vi "Create.vi"   [LabVIEW 2018, in "Toolkit.lvlib" / "Agent.lvclass"]
doc: "Creates a new Agent object that represents a libssh2lv shared library Agent struct. This VI must be called, or executed, before using any other Agent-related VIs. This VI allocates memory within the libssh2lv shared library that must be explicitly deallocated, or freed, at the end of the application using the <B>Destroy</B> VI to avoid memory leaks or running Out-of-Memory (OOM) on a resource contrained system.\n\nAn Agent object represents a connection to a SSH-agent application already running on the local host."
uses:
  Agent.lvclass
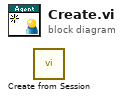
[diagram p0: block diagram]
diagram:
  n1 = call "Create from Session.vi"() -> ()  [unwired: 10 in, 2 out]
